vi "Read UID.vi"(8 "error in":errorcluster, 11 "configuration in":refnum<class "NISE_CEF_serializable configuration.lvclass">) -> (0 "error out":errorcluster, 2 "instance id":string, 3 "configuration out":refnum<class "NISE_CEF_serializable configuration.lvclass">)   [LabVIEW 2014, in "NISE_CEF_serializable configuration.lvclass"]
doc: "Provides the instance name of a given configuration/runtime class pairing. This instance may be used as an identifier to differentiate between configurations. On first call, this instance ID is generated."
uses:
  NISE_CEF_serializable configuration.lvclass
  NISE_CEF_serializable configuration.lvclass/NISE_CEF_serializable configuration.ctl
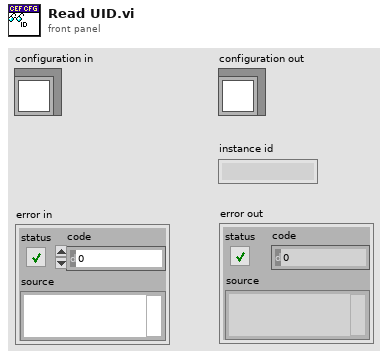
[diagram p1: front panel]
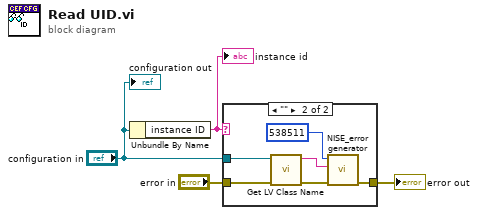
[diagram p0: block diagram]
diagram:
  n1 = Unbundle By Name("configuration in") -> ("instance ID"=w2:string)
  "instance id" <- w2
  n2 = case shown="\"\"" w2 {
    tunnel: [w5 w10] -> w4
    tunnel: "error in" -> [w5 w11]
    tunnel: "configuration in" -> [_ w6]
    frame Default {
    }
    frame "" {
      n3 = call <vilib>:"Get LV Class Name.vi"("error in (no error)"=w11, "object"=w6) -> ("error out"=w8:errorcluster, "class name"=w7:string)  [unwired: 8 in]
      n4 = call "NISE_error generator.vi"("error in"=w8, "append error message"=w7, "error code (0)"=538511) -> ("error out"=w10:errorcluster)  [unwired: 6 in]
    }
  }
  "error out" <- w4
  "configuration out" <- "configuration in"
